vi "test Parse Capabilities Files.vi"(8 "error in (no error)":errorcluster, 11 "TestCase in":refnum<class "SLSC EDS Unit Tests.lvclass">) -> (0 "error out":errorcluster, 3 "TestCase out":refnum<class "SLSC EDS Unit Tests.lvclass">)   [LabVIEW 2020, in "SLSC EDS Unit Tests.lvclass"]
uses:
  SLSC EDS Unit Tests.lvclass
  SLSC EDS API/JSON parsing/EDSjsonStructure.ctl
  SLSC EDS API/JSON parsing/enum.ctl
  SLSC EDS API/JSON parsing/property.ctl
  SLSC EDS API/JSON parsing/command.ctl
  SLSC EDS API/JSON parsing/scale.ctl
  SLSC EDS API/JSON parsing/physicalChannel.ctl
  SLSC EDS API/JSON parsing/register.ctl
  <vilib>/addons/_JKI Toolkits/VI Tester/TestCase.llb/TestCase.lvclass
  C:/Program Files (x86)/National Instruments/LabVIEW 2020/vi.lib/addons/_JKI Toolkits/VI Tester/TestCase.llb/TestCase.lvclass
panel:
  out "Test#":i32
  out "output cluster":cluster{path, bool, bool}
  in  "Empty model":T1
  out "Results (file, not error?, not a valid cap?)":cluster{path, bool, bool}[](array[cluster])
  out "Pass?":bool
  out "Error results":errorcluster[](array[cluster])
  out "Capability results":T1[](array[typedef])
  # "not working\nregisterMap->registers->initialValue"
  # "not working\nregisterMap->registers->initialValue"
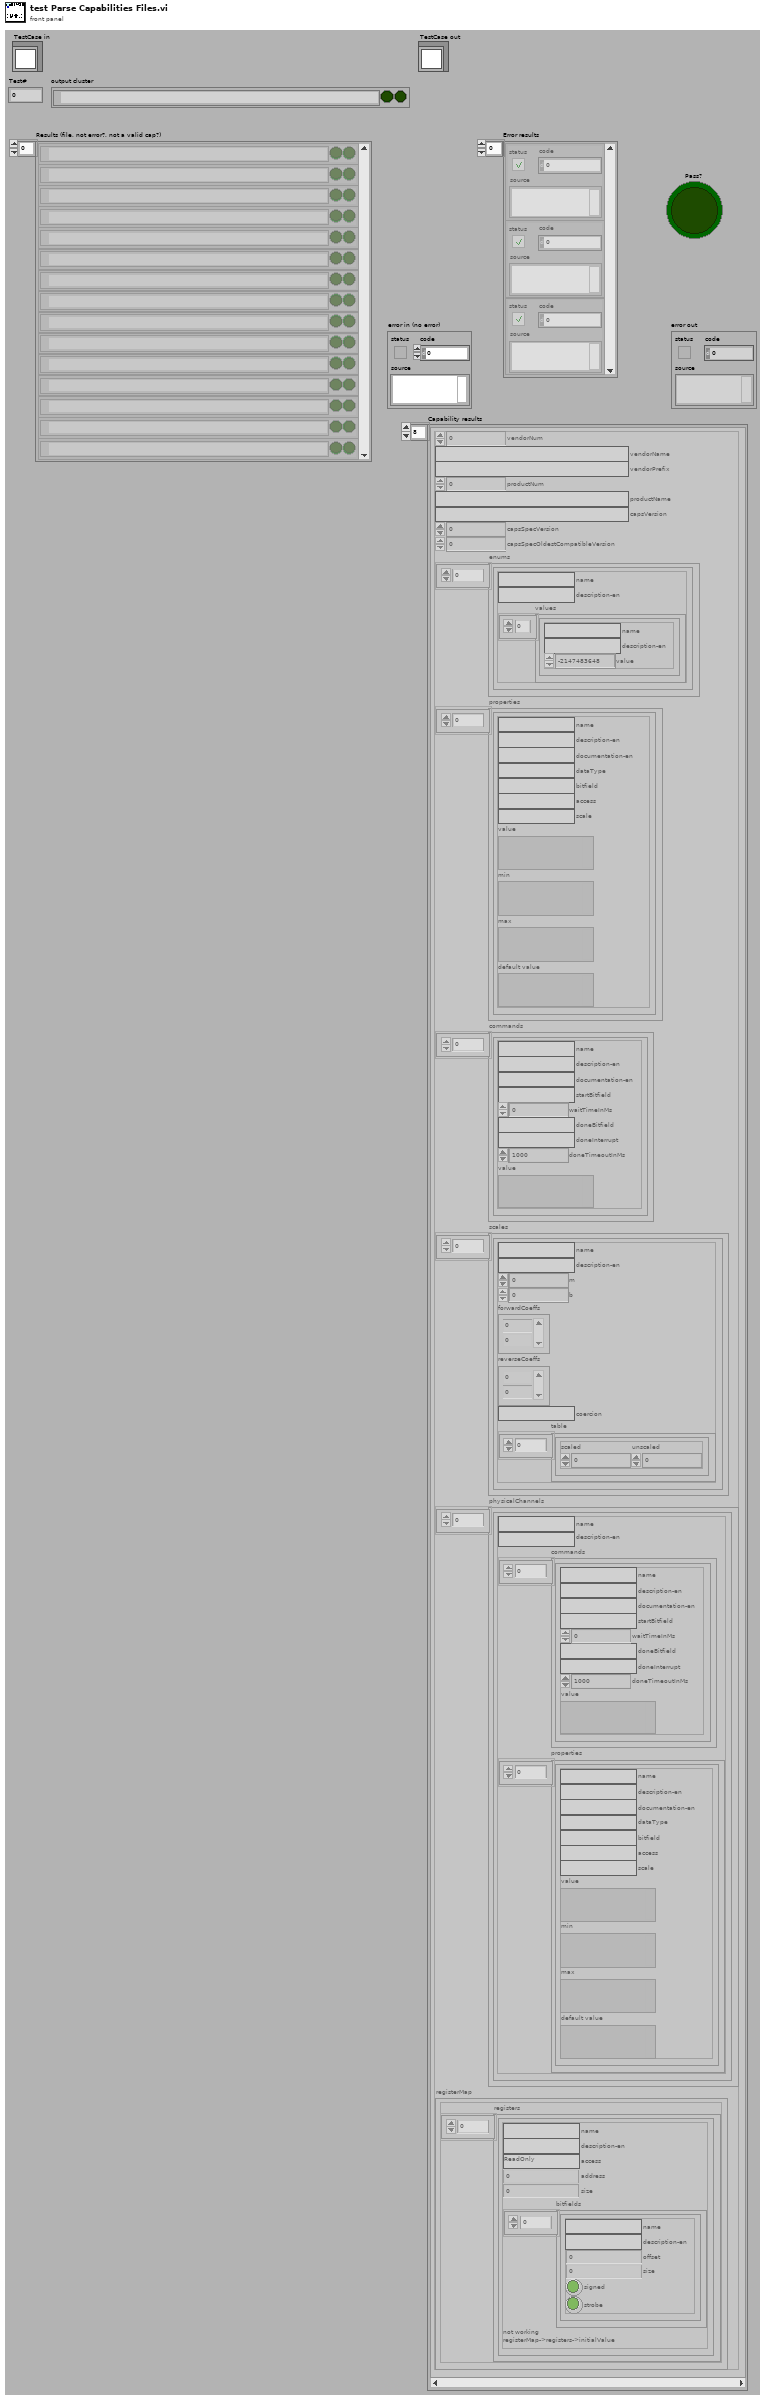
[diagram p1: front panel]
types:
  T1 = typedef "EDSjsonStructure.ctl" = cluster{"vendorNum":u32, "vendorName":string, "vendorPrefix":string, "productNum":u32, "productName":string, "capsVersion":string, "capsSpecVersion":u32, "capsSpecOldestCompatibleVersion":u32, "enums":T2[], "properties":T3[], "commands":T4[], "scales":T5[], "physicalChannels":T6[], "registerMap":cluster{"registers":T7[]}}
  T2 = typedef "enum.ctl" = cluster{"name":string, "description-en":string, "values":cluster{"name":string, "description-en":string, "value":i32}[]}
  T3 = typedef "property.ctl" = cluster{"name":string, "description-en":string, "documentation-en":string, "dataType":string, "bitfield":string, "access":string, "scale":string, "value":variant, "min":variant, "max":variant, "default value":variant}
  T4 = typedef "command.ctl" = cluster{"name":string, "description-en":string, "documentation-en":string, "startBitfield":string, "waitTimeInMs":i32, "doneBitfield":string, "doneInterrupt":string, "doneTimeoutInMs":i32, "value":variant}
  T5 = typedef "scale.ctl" = cluster{"name":string, "description-en":string, "m":dbl, "b":dbl, "forwardCoeffs":dbl[], "reverseCoeffs":dbl[], "coercion":string, "table":cluster{"scaled":dbl, "unscaled":dbl}[]}
  T6 = typedef "physicalChannel.ctl" = cluster{"name":string, "description-en":string, "commands":T4[], "properties":T3[]}
  T7 = typedef "register.ctl" = cluster{"name":string, "description-en":string, "access":string, "address":u32, "size":u32, "bitfields":cluster{"name":string, "description-en":string, "offset":u32, "size":u32, "signed":bool, "strobe":bool}[]}
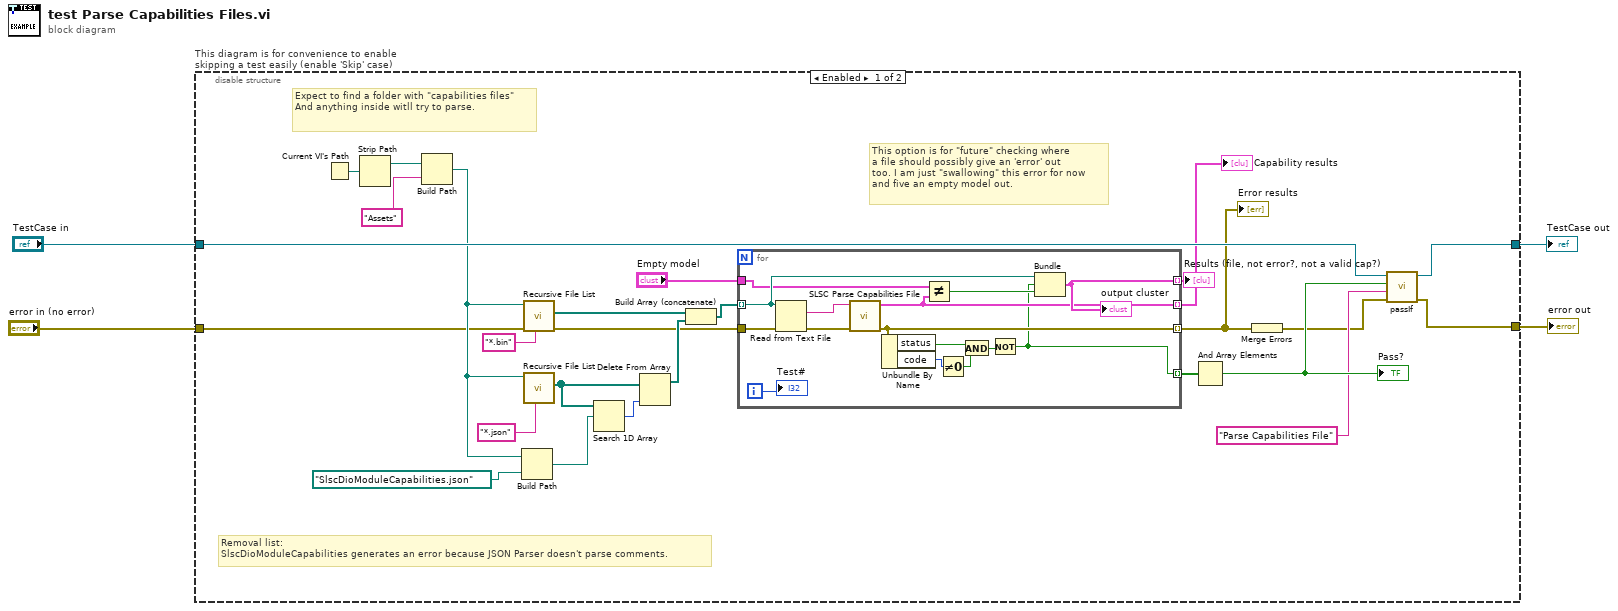
[diagram p0: block diagram]
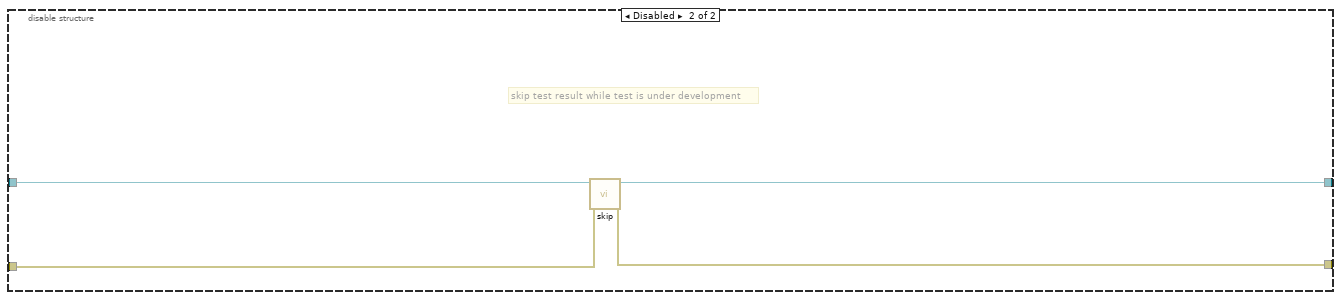
[diagram p2: hidden frame]
diagram:
  n1 = disable-structure "This diagram is for convenience to enable skipping a test easily (enable 'Skip' case)" shown="Enabled" {
    disable-tunnel: "TestCase in" -> [w30 w49]
    disable-tunnel: [w29 w47] -> w1
    disable-tunnel: [w28 w48] -> w3
    disable-tunnel: "error in (no error)" -> [w11 w46]
    frame Enabled {
      # "This option is for \"future\" checking where\na file should possibly give an 'error' out \ntoo. I am just \"swallowing\" this error for now\nand five an empty model out."
      # "Expect to find a folder with \"capabilities files\" \nAnd anything inside witll try to parse."
      # "Removal list:\nSlscDioModuleCapabilities generates an error because JSON Parser doesn't parse comments."
      n2 = Current VI's Path() -> (path=w27:path)
      n3 = Strip Path(path=w27) -> (stripped path=w16:path)  [unwired: 1 out]
      n4 = Build Path(base path=w16, name or relative path="Assets") -> (appended path=w13:path)
      n5 = Build Path(base path=w13, name or relative path=path "SlscDioModuleCapabilities.json" ("element")) -> (appended path=w12:path)
      n6 = call <vilib>:"Recursive File List.vi"("pattern"="*.bin", "error in (no error)"=w11, "Folder Path"=w13) -> ("error out"=w9:errorcluster, "All Files in Dir"=w25:path[])  [unwired: 4 in, 3 out]
      n7 = call <vilib>:"Recursive File List.vi"("pattern"="*.json", "Folder Path"=w13) -> ("All Files in Dir"=w19:path[])  [unwired: 5 in, 4 out]
      n8 = Search 1D Array(1D array=w19, element=w12) -> (index of element=w21:i32)  [unwired: 1 in]
      n9 = Delete From Array(array=w19, index=w21) -> (array with subset deleted=w17:path[])  [unwired: 1 in, 1 out]
      n10 = Build Array (concatenate)(w25, w17) -> (w23:path[])
      n11 = for {
        tunnel: w23 -> [w37] mode=indexing
        tunnel: [w35] -> w24 mode=indexing
        tunnel: [w31] -> w20 mode=indexing
        tunnel: [w40] -> w8 mode=indexing
        tunnel: w9 -> [w39]
        tunnel: [w36] -> w6 mode=indexing
        tunnel: "Empty model" -> [w34]
        i -> [w32]
        n12 = Read from Text File(file (use dialog)=w37, error in=w39) -> (text=w45:string, error out=w44:errorcluster)  [unwired: 2 in, 2 out]
        n13 = call "SLSC Parse Capabilities File.vi"("error in"=w44, "module capabilities JSON string"=w45) -> ("error out"=w40:errorcluster, "SLSC EDS module"=w35:T1)  [unwired: 7 in, 1 out]
        n14 = Unbundle By Name(w40) -> ("status"=w43:bool, "code"=w42:i32)
        n15 = Not Equal?(x=w34, y=w35) -> (x != y?=w33:bool)
        n16 = Not Equal To 0?(x=w42) -> (x != 0?=w41:bool)
        n17 = And(x=w43, y=w41) -> (x .and. y?=w38:bool)
        n18 = Not(x=w38) -> (.not. x?=w31:bool)
        n19 = Bundle(w37, w31, w33) -> (w36:cluster{path, bool, bool})  [unwired: 1 in]
        "output cluster" <- w36
        "Test#" <- w32
      }
      "Capability results" <- w24
      "Error results" <- w8
      "Results (file, not error?, not a valid cap?)" <- w6
      n20 = And Array Elements(Boolean array=w20) -> (logical AND=w18:bool)
      "Pass?" <- w18
      n21 = Merge Errors(w8) -> (w7:errorcluster)
      n22 = call-dynamic "passIf.vi"("error in (no error)"=w7, "message (\"\")"="Parse Capabilities File" ("message (\"\")"), "pass"=w18, "TestCase in"=w30) -> ("error out"=w28:errorcluster, "TestCase out"=w29:refnum<class "SLSC EDS Unit Tests.lvclass">)  [unwired: 6 in]
    }
    frame Disabled {
      # "skip test result while test is under development"
      n23 = call <vilib>:"skip.vi"("error in (no error)"=w46, "TestCase in"=w49) -> ("error out"=w48:errorcluster, "TestCase out"=w47:refnum<class "SLSC EDS Unit Tests.lvclass">)  [unwired: 8 in]
    }
  }
  "error out" <- w3
  "TestCase out" <- w1
